vi "RFH-common_format_to_element_map.vi"(10 "Common Format":T1) -> (2 "Element map":map{dbl, T2}(c390))   [LabVIEW 2020, in "RFH-Reflection_File_Handler.lvlib"]
doc: "Converts a Common Format cluster into a map from frequency to data point."
uses:
  RFH-Reflection_File_Handler.lvlib
  RFH-common_data_format_element.ctl
  RFH-common_data_format.ctl
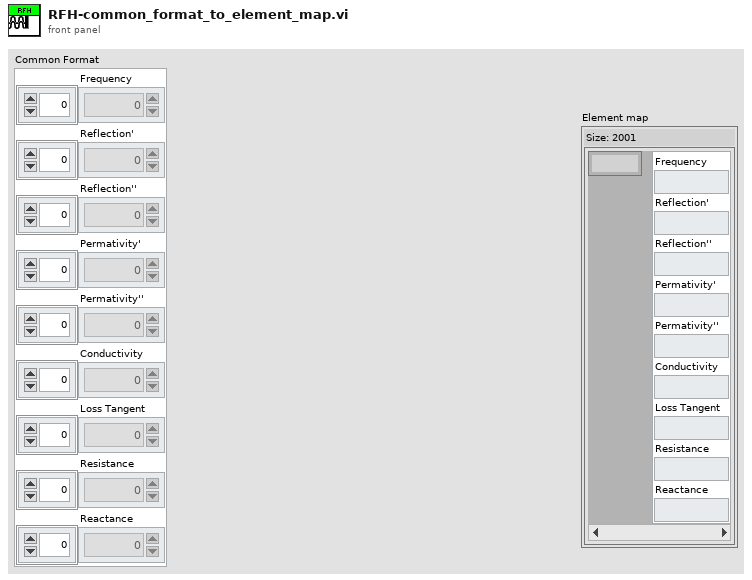
[diagram p1: front panel]
types:
  T1 = typedef "RFH-Reflection_File_Handler.lvlib/RFH-common_data_format.ctl" = cluster{"Frequency":dbl[], "Reflection'":dbl[], "Reflection''":dbl[], "Permativity'":dbl[], "Permativity''":dbl[], "Conductivity":dbl[], "Loss Tangent":dbl[], "Resistance":dbl[], "Reactance":dbl[]}
  T2 = typedef "RFH-Reflection_File_Handler.lvlib/RFH-common_data_format_element.ctl" = cluster{"Frequency":dbl, "Reflection'":dbl, "Reflection''":dbl, "Permativity'":dbl, "Permativity''":dbl, "Conductivity":dbl, "Loss Tangent":dbl, "Resistance":dbl, "Reactance":dbl}
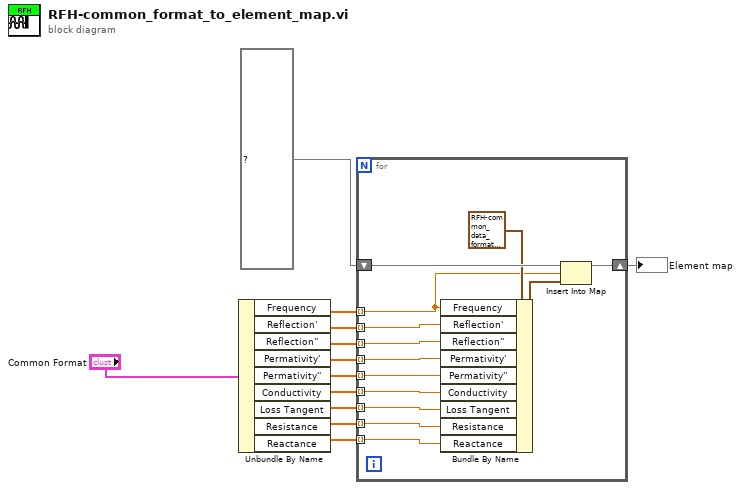
[diagram p0: block diagram]
diagram:
  n1 = Unbundle By Name("Common Format") -> ("Frequency"=w5:dbl[], "Reflection'"=w6:dbl[], "Reflection''"=w7:dbl[], "Permativity'"=w8:dbl[], "Permativity''"=w9:dbl[], "Conductivity"=w11:dbl[], "Loss Tangent"=w12:dbl[], "Resistance"=w2:dbl[], "Reactance"=w1:dbl[])
  n2 = for {
    shift-right: [w24] -> w4
    shift-left: map{dbl, T2} {} ("map") -> [w25]
    tunnel: w12 -> [w21] mode=indexing
    tunnel: w11 -> [w20] mode=indexing
    tunnel: w9 -> [w19] mode=indexing
    tunnel: w8 -> [w18] mode=indexing
    tunnel: w7 -> [w17] mode=indexing
    tunnel: w6 -> [w16] mode=indexing
    tunnel: w5 -> [w15] mode=indexing
    tunnel: w2 -> [w14] mode=indexing
    tunnel: w1 -> [w13] mode=indexing
    n3 = Bundle By Name(cluster=T2 {"Frequency"=0.0, "Reflection'"=0.0, "Reflection''"=0.0, "Permativity'"=0.0, "Permativity''"=0.0, "Conductivity"=0.0, "Loss Tangent"=0.0, "Resistance"=0.0, "Reactance"=0.0} ("Common Format"), "Frequency"=w15, "Reflection'"=w16, "Reflection''"=w17, "Permativity'"=w18, "Permativity''"=w19, "Conductivity"=w20, "Loss Tangent"=w21, "Resistance"=w14, "Reactance"=w13) -> (w22:T2)
    n4 = Insert Into Map(map in=w25, key=w15, value=w22) -> (map out=w24:map{dbl, T2})  [unwired: 2 out]
  }
  "Element map" <- w4
